vi "Replace Parameter Cluster.vi"(8 "error in":errorcluster, 10 "Parameter Mode":T1, 11 "Virtual Instrument in":refnum<class "Virtual Instrument.lvclass">) -> (0 "error out":errorcluster, 3 "Virtual Instrument out":refnum<class "Virtual Instrument.lvclass">)   [LabVIEW 2026, in "Virtual Instrument.lvclass"]
doc: "This VI replaces the input/output parameter cluster of the current VI by the specific type definition. The type definition must be created beforehand."
uses:
  Virtual Instrument.lvclass
  Type Definitions/Parameter Mode--enum.ctl
  <vilib>/Utility/traverseref.llb/TRef TravTarget.ctl
  Virtual Instrument.lvclass/Virtual Instrument.ctl
  LabVIEW File/LabVIEW File.lvclass/LabVIEW File.ctl
  LabVIEW File/Read VI Reference.vi
  LabVIEW File/Read Name.vi
  <userlib>/_OpenG.lib/file/file.llb/File Exists - Scalar__ogtk.vi
  <userlib>/_OpenG.lib/file/file.llb/openg_file.lvlib
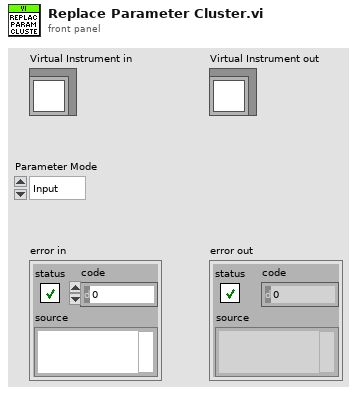
[diagram p1: front panel]
types:
  T1 = typedef "Parameter Mode--enum.ctl" = enum16{"Input", "Output"}
  T2 = typedef "TRef TravTarget.ctl" = enum16{"FP", "BD", "Other"}
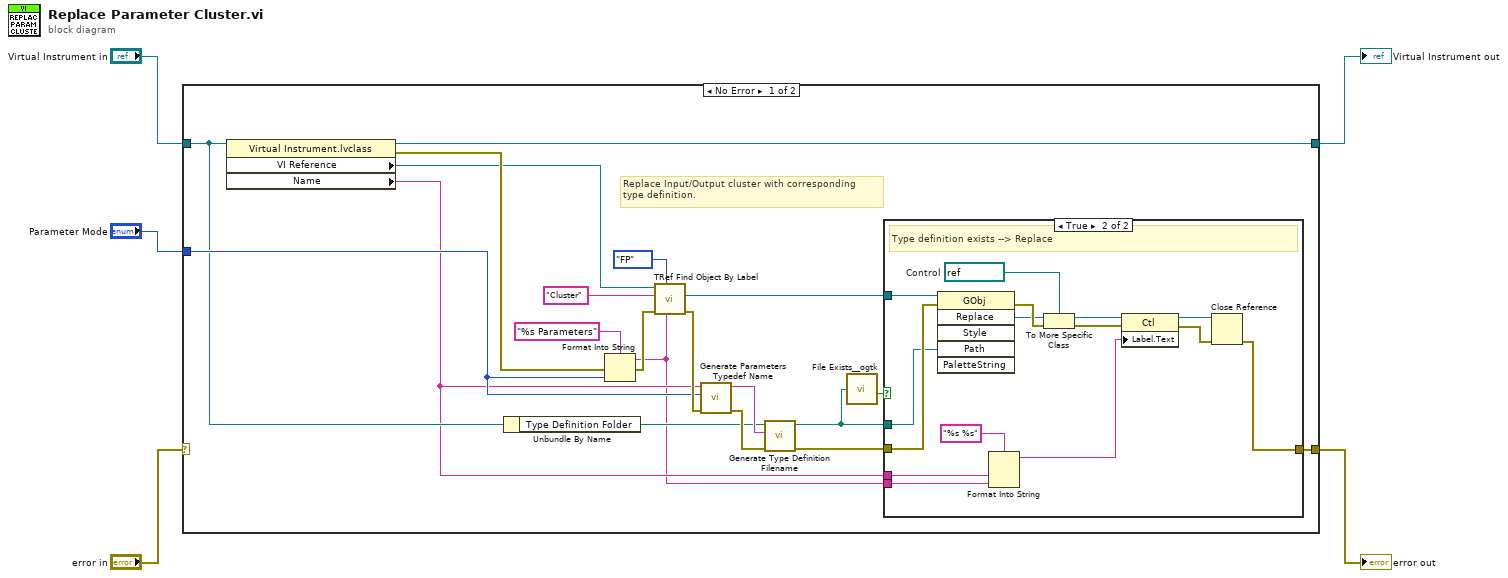
[diagram p0: block diagram]
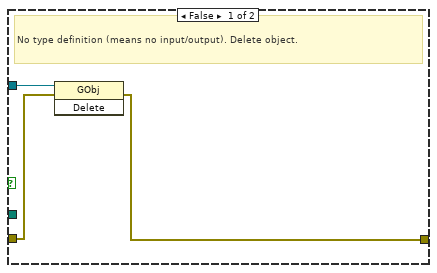
[diagram p2: hidden frame]
diagram:
  n1 = case shown="No Error" "error in" {
    selector: "error in" -> [_ w45]
    tunnel: [w21 w45] -> w4
    tunnel: [w12 w44] -> w2
    tunnel: "Virtual Instrument in" -> [w10 w44]
    tunnel: "Parameter Mode" -> [w16 _]
    frame No Error {
      # "Replace Input/Output cluster with corresponding\ntype definition."
      n2 = property on="Property Node" class="Virtual Instrument.lvclass"(reference=w10) -> (reference out=w12:refnum<class "Virtual Instrument.lvclass">, error out=w20:errorcluster, "VI Reference"=w11:refnum<vi>, "Name"=w7:string)  [unwired: 1 in]
      n3 = Unbundle By Name(w10) -> ("Type Definition Folder"=w9:path)
      n4 = Format Into String(format string="%s Parameters", error in=w20, w16) -> (resulting string=w6:string, error out=w25:errorcluster)  [unwired: 1 in]
      n5 = call <vilib>:"TRef Find Object By Label.vi"("Label"=w6, "Traverse Target"=TRef_TravTarget."FP", "error in (no error)"=w25, "Class Name"="Cluster", "VI Ref"=w11) -> ("error out"=w24:errorcluster, "Found Obj Ref"=w8:refnum<vi>)  [unwired: 3 in, 2 out]
      n6 = call "Generate Parameters Typedef Name.vi"("error in"=w24, "Parameter Mode"=w16, "VI Name"=w7) -> ("error out"=w23:errorcluster, "Type Definition Name"=w15:string)  [unwired: 7 in]
      n7 = call "Generate Type Definition Filename.vi"("error in"=w23, "Name"=w15, "Path"=w9) -> ("error out"=w22:errorcluster, "Typedef Path"=w14:path)  [unwired: 7 in]
      n8 = call-poly <userlib>:"File Exists__ogtk.vi"("file path"=w14) -> ("exists"=w13:bool)  [unwired: 6 in, 1 out]
      n9 = case shown="True" w13 {
        tunnel: w22 -> [w27 w43]
        tunnel: [w28 w42] -> w21
        tunnel: w8 -> [w26 w38]
        tunnel: w14 -> [_ w37]
        tunnel: w7 -> [_ w31]
        tunnel: w6 -> [_ w30]
        frame False {
          # "No type definition (means no input/output). Delete object."
          n10 = invoke on="Invoke Node" class="GObj" method="Delete"(reference=w26, error in=w27) -> (error out=w28:errorcluster)  [unwired: 1 in, 2 out]
        }
        frame True {
          w36 = refnum<vi> refnum  # Control
          # "Type definition exists --> Replace"
          n11 = invoke on="Invoke Node" class="GObj" method="Replace"(reference=w38, error in=w43, "Path"=w37) -> (error out=w41:errorcluster, "Replace"=w35:refnum<vi>)  [unwired: 3 in, 4 out]
          n12 = Format Into String(format string="%s %s", w31, w30) -> (resulting string=w29:string)  [unwired: 2 in, 1 out]
          n13 = To More Specific Class(target class=w36, reference=w35, error in=w41) -> (specific class reference=w34:refnum<vi>, error out=w40:errorcluster)
          n14 = property class="Ctl"(reference=w34, error in=w40, "Label.Text"=w29) -> (reference out=w33:refnum<vi>, error out=w39:errorcluster)
          n15 = Close Reference(reference=w33, error in (no error)=w39) -> (error out=w42:errorcluster)
        }
      }
    }
    frame Error {
    }
  }
  "error out" <- w4
  "Virtual Instrument out" <- w2
